vi "Une acqui compteur.vi"(4 "entrées":bool[][](array[boolean])=[[FALSE, TRUE, FALSE, FALSE, TRUE, FALSE, FALSE, FALSE, FALSE, FALSE, FALSE, TRUE, FALSE, FALSE, FALSE, FALSE, FALSE, FALSE, FALSE, FALSE, FALSE, FALSE], [FALSE, FALSE, FALSE, FALSE, FALSE, FALSE, TRUE, FALSE, FALSE, TRUE, FALSE, FALSE, TRUE, FALSE, FALSE, FALSE, FALSE, FALSE, FALSE, FALSE, FALSE, FALSE]], 5 "BF2 i-1":bool[](array[boolean]), 6 "BF1 i-1":bool[](array[boolean]), 7 "s-1":bool[](array[boolean]), 8 "Valeurs compteur i-1":dbl[](array[numeric]) format="%.2f") -> (0 "BF2 i":bool[](array[boolean]), 1 "BF1 i":bool[](array[boolean]), 2 "S":bool[](array[boolean]), 3 "Valeur compteur":dbl[](array[numeric]) format="%.2f")   [LabVIEW 2022 SP3]
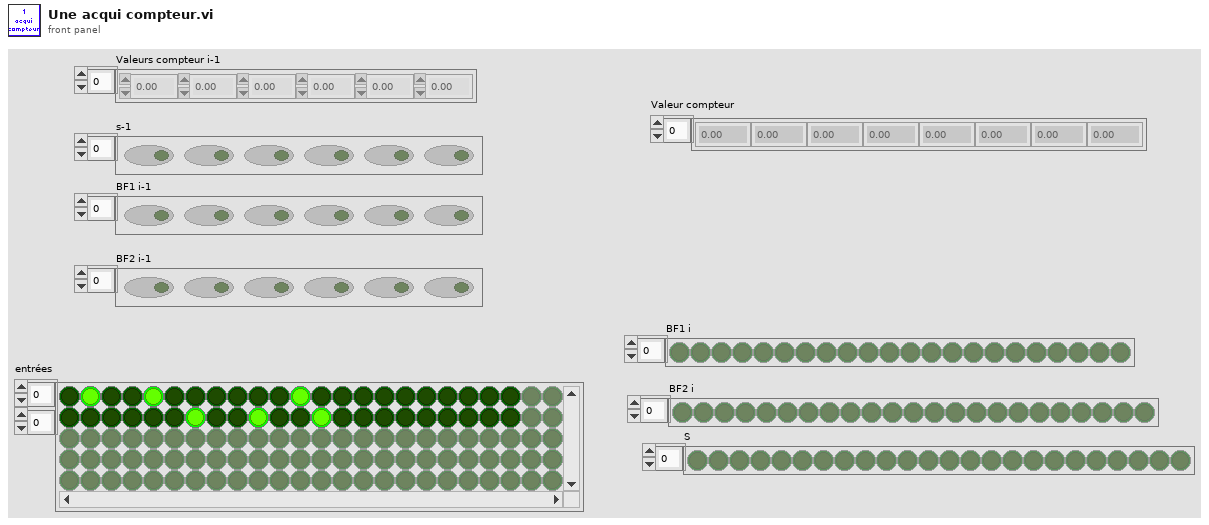
[diagram p1: front panel]
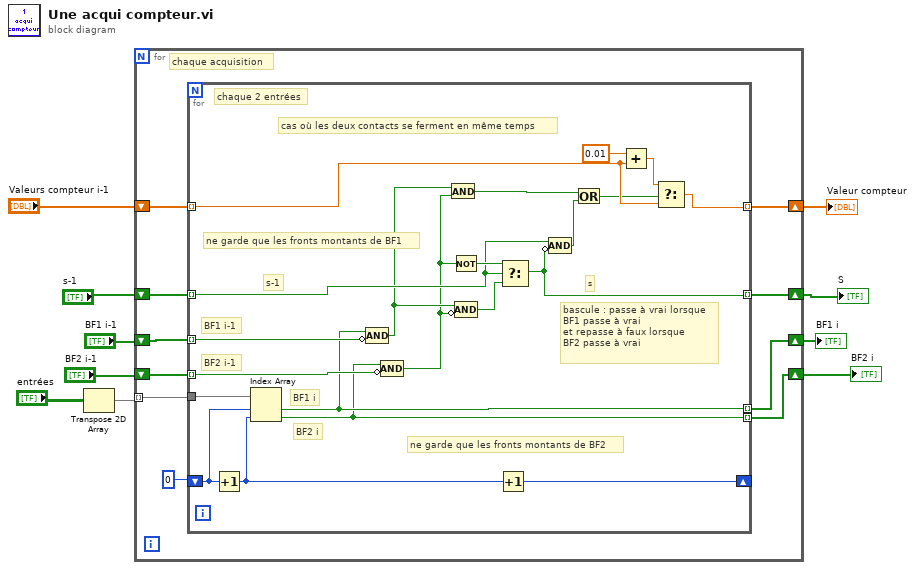
[diagram p0: block diagram]
diagram:
  n1 = Transpose 2D Array(2D array="entrées") -> (transposed array=w10:bool[][])
  n2 = for {
    tunnel: w10 -> [w17] mode=indexing
    shift-right: [w18] -> w8
    shift-left: "Valeurs compteur i-1" -> [w20]
    shift-right: [w15] -> w2
    shift-left: "BF1 i-1" -> [w19]
    shift-right: [w14] -> w1
    shift-left: "BF2 i-1" -> [w16]
    shift-right: [w12] -> w3
    shift-left: "s-1" -> [w13]
    # "chaque acquisition"
    n3 = for {
      tunnel: w17 -> [w40]
      tunnel: w20 -> [w37] mode=indexing
      tunnel: w19 -> [w41] mode=indexing
      tunnel: [w38] -> w18 mode=indexing
      tunnel: w16 -> [w39] mode=indexing
      tunnel: [w27] -> w15 mode=indexing
      tunnel: [w26] -> w14 mode=indexing
      tunnel: w13 -> [w31] mode=indexing
      tunnel: [w28] -> w12 mode=indexing
      shift-right: [w22] -> _
      shift-left: 0 -> [w24]
      # "bascule : passe à vrai lorsque \nBF1 passe à vrai \net repasse à faux lorsque \nBF2 passe à vrai"
      # "cas où les deux contacts se ferment en même temps"
      # "ne garde que les fronts montants de BF1"
      # "ne garde que les fronts montants de BF2"
      # "s"
      # "s-1"
      # "BF2 i"
      # "BF1 i"
      # "BF2 i-1"
      # "BF1 i-1"
      # "chaque 2 entrées"
      n4 = Increment(x=w24) -> (x+1=w23:i32)
      n5 = Index Array(array=w40, index #1=w24, index #2=w23) -> (element #1=w27:bool, element #2=w26:bool)
      n6 = Compound Arithmetic op=AND ("Opérateur arithmétique")(w27, invert w41) -> (w30:bool)
      n7 = Compound Arithmetic op=AND ("Opérateur arithmétique")(w26, invert w39) -> (w29:bool)
      n8 = And(x=w30, y=w29) -> (x .and. y?=w34:bool)
      n9 = Not(x=w29) -> (.not. x?=w35:bool)
      n10 = Compound Arithmetic op=AND ("Opérateur arithmétique")(w30, invert w29) -> (w36:bool)
      n11 = Increment(x=w23) -> (x+1=w22:i32)
      n12 = Select(t=w35, s=w31, f=w36) -> (s? t:f=w28:bool)
      n13 = Compound Arithmetic op=AND ("Opérateur arithmétique")(w31, invert w28) -> (w32:bool)
      n14 = Or(x=w34, y=w32) -> (x .or. y?=w25:bool)
      n15 = Add(x=0.01, y=w37) -> (x+y=w33:dbl)
      n16 = Select(t=w33, s=w25, f=w37) -> (s? t:f=w38:dbl)
    }
  }
  "Valeur compteur" <- w8
  "S" <- w3
  "BF1 i" <- w2
  "BF2 i" <- w1
